vi "FuncVI-QueueGetAll.vi"(5 "InstanceRef":T2, 9 "arg list":T1[](array[typedef]) {"num" format="%.2f"}) -> (0 "error out":bool, 3 "result":T1 {"num" format="%.2f"})   [LabVIEW 2021]
doc: "::: CalcExpress Toolkit :::\nCopyright (c) 2000-2026 Konstantin Shifershteyn. All rights reserved."
uses:
  cetypes.llb/CalcExpress Function Argument Info.ctl
  cetypes.llb/CalcExpress Instance RefNum.ctl
panel:
  in  "max arg num":i32=1
  in  "min arg num":i32=1
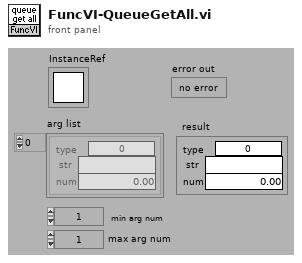
[diagram p1: front panel]
types:
  T1 = typedef "CalcExpress Function Argument Info.ctl" = cluster{"type":u32, "str":string, "num":dbl}
  T2 = typedef "CalcExpress Instance RefNum.ctl" = refnum<k1>
  T3 = enum32{"String", "DBL Number", "identifier", "1D Array of DBL", "2D Array of DBL", "CDB Number", "1D Array of CDB", "2D Array of CDB", "1D Array of String", "2D Array of String", "Unknown data type"}
  T4 = cluster{"data type":enum32{"String", "DBL Number", "identifier", "1D Array of DBL", "2D Array of DBL", "CDB Number", "1D Array of CDB", "2D Array of CDB", "1D Array of String", "2D Array of String", "Unknown data type"}, "data string":string, dbl}
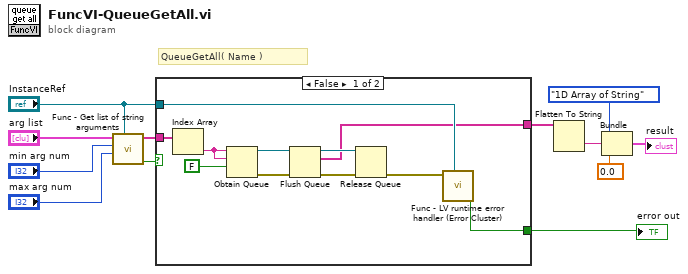
[diagram p0: block diagram]
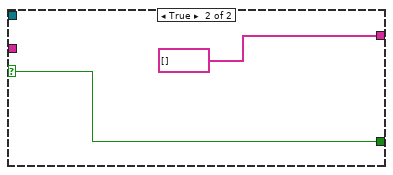
[diagram p2: hidden frame]
diagram:
  # "QueueGetAll( Name )"
  n1 = call "Func - Get list of string arguments.vi"("InstanceRef"="InstanceRef", "max arg num"="max arg num", "min arg num"="min arg num", "arg list"="arg list") -> ("error out"=w4:bool, "val list"=w11:string[])  [unwired: 4 in]
  n2 = case shown="False" w4 {
    selector: w4 -> [_ w24]
    tunnel: w11 -> [w23 _]
    tunnel: [w14 string[] [] ("elements")] -> w6
    tunnel: "InstanceRef" -> [w22 _]
    tunnel: [w21 w24] -> w3
    frame False {
      n3 = Index Array(array=w23) -> (element=w16:string)  [unwired: 1 in]
      n4 = Obtain Queue(name (unnamed)=w16, element data type=w16, create if not found? (T)=FALSE) -> (queue out=w20:refnum<queue>, error out=w18:errorcluster)  [unwired: 2 in, 1 out]
      n5 = Flush Queue(queue=w20, error in (no error)=w18) -> (queue out=w19:refnum<queue>, remaining elements=w14:string[], error out=w17:errorcluster)
      n6 = Release Queue(queue=w19, error in (no error)=w17) -> (error out=w13:errorcluster)  [unwired: 1 in, 2 out]
      n7 = call "Func - LV runtime error handler (Error Cluster).vi"("InstanceRef"=w22, "LabVIEW error"=w13) -> ("error out"=w21:bool)  [unwired: 4 in, 3 out]
    }
    frame True {
    }
  }
  "error out" <- w3
  n8 = Flatten To String(anything=w6) -> (data string=w5:string)  [unwired: 3 in, 2 out]
  n9 = Bundle("data type"=T3."1D Array of String", "data string"=w5, 0.0) -> (→"result":T4)  [unwired: 1 in]
